vi "Read_Image(Batch).vi"(5 "mBatch":i32, 6 "PreProcessing_Options":T1={"DS_Name"="", "Input_Dims"={"C"=3, "H"=224, "W"=224}, "Cropping"={"Left"=0.0, "Top"=0.0, "Right"=1.0, "Bottom"=1.0}, "Interpolation Type"=1, "MultiStage_ReSample?"=FALSE, "Dataset_Stats"={"means"={"R"=0.5385, "G"=0.5348, "B"=0.551}, "stds"={"R"=0.3673, "G"=0.3673, "B"=0.3505}}} {"Dataset_Stats"."stds"."R" format="%#_3g"; "Dataset_Stats"."stds"."G" format="%#_3g"; "Dataset_Stats"."stds"."B" format="%#_3g"; "Dataset_Stats"."means"."R" format="%#_3g"; "Dataset_Stats"."means"."G" format="%#_3g"; "Dataset_Stats"."means"."B" format="%#_3g"; "Interpolation Type" items=["Zero Order", "Bi-Linear", "Quadratic", "Cubic Spline"]}, 8 "error in":errorcluster, 9 "index":i32, 11 "File_Paths":path[][](array[path])) -> (0 "error out":errorcluster, 2 "dT_Img_Read":dbl format="%0.2f", 3 "Image(Batch) Out":sgl[][][][](array[numeric]))   [LabVIEW 2020]
uses:
  <vilib>/Ngene/DeepLTK Anomaly Detection Addon/Toolkit/API/Controls/NNPC_PreProcessing_Options.ctl
  <vilib>/Ngene/Deep Learning Toolkit/Toolkit/NN_Data/API/NN_Dims(C,H,W).ctl
  <vilib>/Ngene/DeepLTK Anomaly Detection Addon/Toolkit/API/Controls/Crop_CFG.ctl
  <vilib>/Ngene/DeepLTK Anomaly Detection Addon/Toolkit/API/Controls/NNPC_DS_Stats.ctl
  <vilib>/Ngene/DeepLTK Anomaly Detection Addon/Toolkit/API/Controls/Image_Stats_RGB.ctl
  <vilib>/Analysis/baseanly.llb/Mean (DBL).vi
  <vilib>/Analysis/NI_AALBase.lvlib
  <vilib>/Ngene/Deep Learning Toolkit/Toolkit/Deep_Learning_Toolkit_by_Ngene.lvlib
  <vilib>/Ngene/DeepLTK Anomaly Detection Addon/Toolkit/DeepLTK_Anomaly_Detection_Addon.lvlib
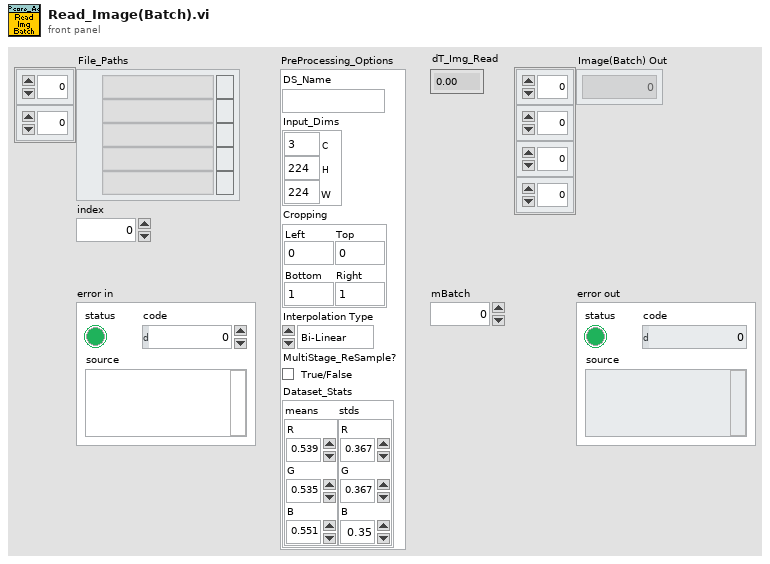
[diagram p1: front panel]
types:
  T1 = typedef "DeepLTK_Anomaly_Detection_Addon.lvlib/NNPC_PreProcessing_Options.ctl" = cluster{"DS_Name":string, "Input_Dims":T2, "Cropping":T3, "Interpolation Type":u32, "MultiStage_ReSample?":bool, "Dataset_Stats":T4}
  T2 = typedef "Deep_Learning_Toolkit_by_Ngene.lvlib/NN_Dims(C,H,W).ctl" = cluster{"C":i32, "H":i32, "W":i32}
  T3 = typedef "DeepLTK_Anomaly_Detection_Addon.lvlib/Crop_CFG.ctl" = cluster{"Left":sgl, "Top":sgl, "Right":sgl, "Bottom":sgl}
  T4 = typedef "DeepLTK_Anomaly_Detection_Addon.lvlib/NNPC_DS_Stats.ctl" = cluster{"means":T5, "stds":T5}
  T5 = typedef "DeepLTK_Anomaly_Detection_Addon.lvlib/Image_Stats_RGB.ctl" = cluster{"R":sgl, "G":sgl, "B":sgl}
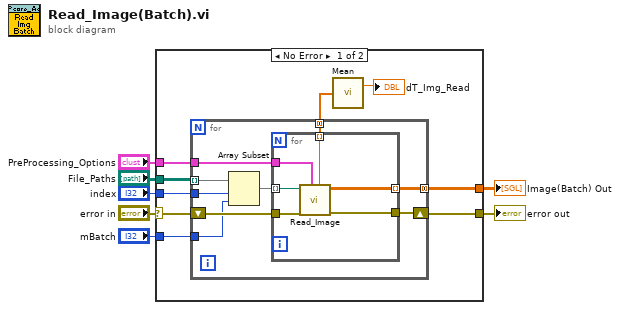
[diagram p0: block diagram]
diagram:
  n1 = case shown="No Error" "error in" {
    selector: "error in" -> [w10 w32]
    tunnel: [w16 _] -> w7
    tunnel: [w15 w32] -> w6
    tunnel: "File_Paths" -> [w14 _]
    tunnel: "index" -> [w13 _]
    tunnel: "mBatch" -> [w9 _]
    tunnel: "PreProcessing_Options" -> [w8 _]
    frame No Error {
      n2 = for {
        tunnel: [w24] -> w12 mode=concatenating
        tunnel: w14 -> [w20] mode=indexing
        tunnel: [w23] -> w16 mode=concatenating
        shift-right: [w22] -> w15
        shift-left: w10 -> [w25]
        tunnel: w13 -> [w19]
        tunnel: w9 -> [w18]
        tunnel: w8 -> [w17]
        n3 = Array Subset(array=w20, index=w19, length=w18) -> (w21:path[])
        n4 = for {
          tunnel: w25 -> [w31]
          tunnel: [w30] -> w24 mode=indexing
          tunnel: w21 -> [w29] mode=indexing
          tunnel: [w28] -> w23 mode=indexing
          tunnel: [w27] -> w22
          tunnel: w17 -> [w26]
          n5 = call "Read_Image.vi"("PreProcessing_Options"=w26, "error in"=w31, "Img Path"=w29) -> ("error out"=w27:errorcluster, "Image Out (Preproc)"=w28:sgl[][][], "dT_Img_Read"=w30:dbl)  [unwired: 3 in, 3 out]
        }
      }
      n6 = call-poly <vilib>:"Mean.vi"("X"=w12) -> ("mean"=→"dT_Img_Read":dbl)  [unwired: 1 out]
    }
    frame Error {
    }
  }
  "Image(Batch) Out" <- w7
  "error out" <- w6
